vi "put box.vi"(2 "error in (no error)":errorcluster, 3 "¬Ö¼Æ":i32) -> (0 "error out":errorcluster)   [LabVIEW 2019]
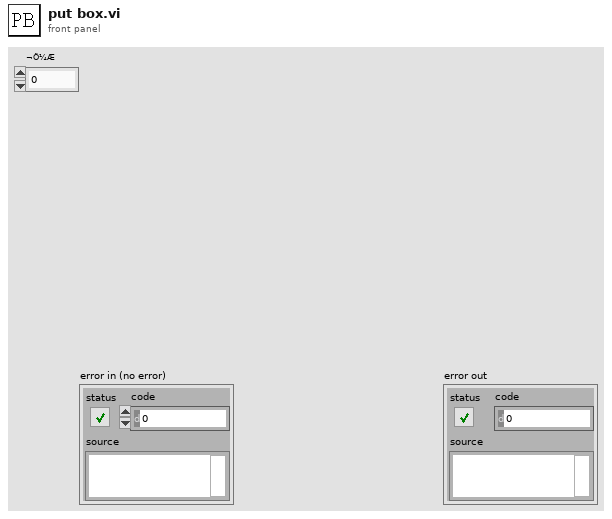
[diagram p1: front panel]
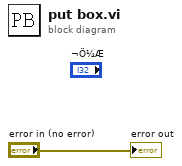
[diagram p0: block diagram]
diagram:
  "error out" <- "error in (no error)"
